vi "Error_to_string.vi"(8 "error in (no error)":errorcluster, 11 "spreadsheet string in":string) -> (3 "spreadsheet string out":string)   [LabVIEW 2020]
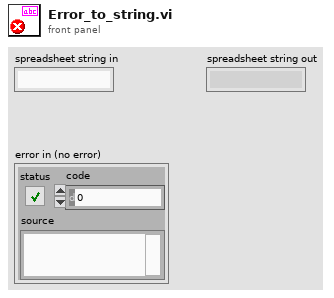
[diagram p1: front panel]
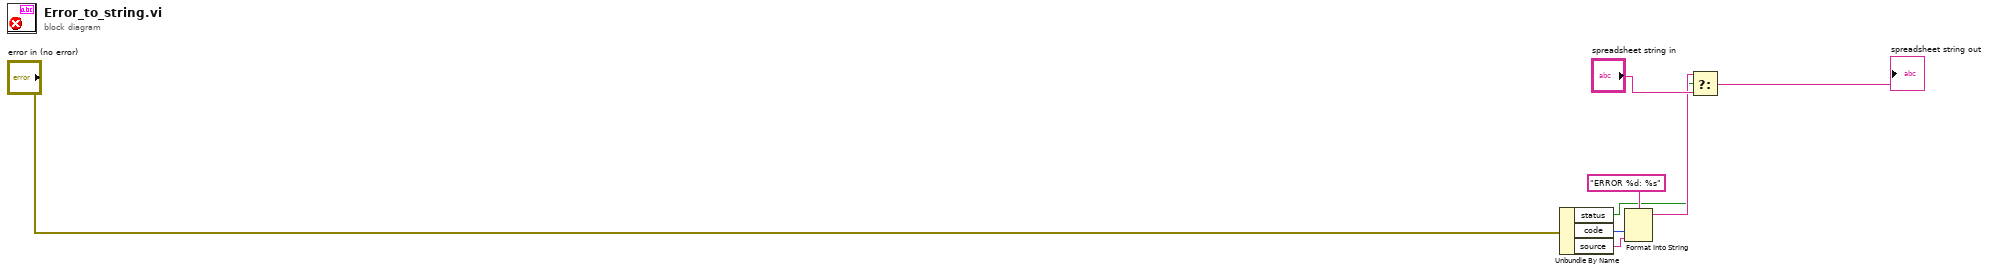
[diagram p0: block diagram]
diagram:
  n1 = Unbundle By Name("error in (no error)") -> ("status"=w2:bool, "code"=w4:i32, "source"=w5:string)
  n2 = Format Into String(format string="ERROR %d: %s", w4, w5) -> (resulting string=w6:string)  [unwired: 2 in, 1 out]
  n3 = Select(t=w6, s=w2, f="spreadsheet string in") -> (s? t:f=→"spreadsheet string out":string)
